vi "Should Stop.vi"(7 "Actor in":refnum<class "Actor.lvclass">, 8 "Error in":errorcluster, 10 "Msg Output":refnum<class "Msg Output.lvclass">) -> (0 "Error out":errorcluster, 2 "Stop":bool, 5 "Actor out":refnum<class "Actor.lvclass">)   [LabVIEW 2020, in "jettl.lvlib"]
uses:
  jettl.lvlib
  Actor/Actor.lvclass
  Msg Output/Msg Output.lvclass
  Msg/Msg.lvclass
  Teardown Location.ctl
  Stop jettl Msg/Stop/Call.vi
  Attributes/Attributes.lvclass
  Transport/Transport.lvclass
  Stop jettl Msg/Stop/Stop.lvlib
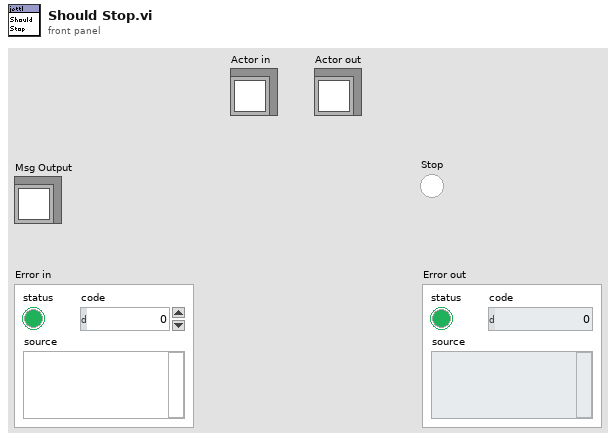
[diagram p1: front panel]
types:
  T1 = typedef "jettl.lvlib/Teardown Location.ctl" = enum16{"Starting", "Should Stop"}
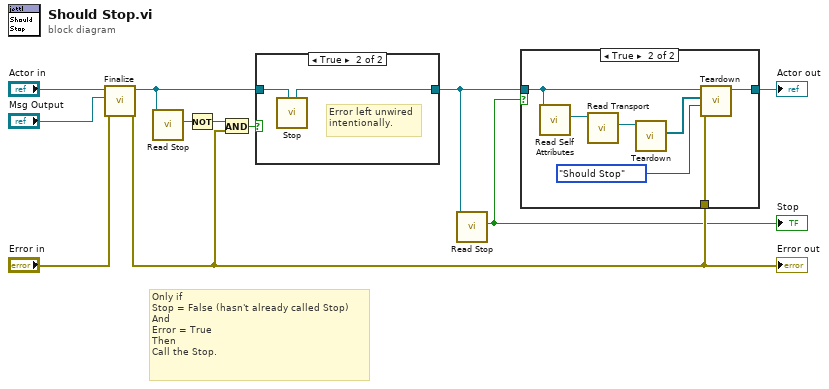
[diagram p0: block diagram]
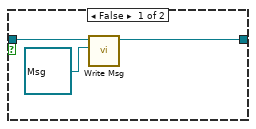
[diagram p3: hidden frame]
diagram:
  # "Only if\nStop = False (hasn't already called Stop)\nAnd\nError = True\nThen\nCall the Stop."
  n1 = call-dynamic "Finalize.vi"("Error in"="Error in", "Msg Output"="Msg Output", "Actor in"="Actor in") -> ("Error out"=w2:errorcluster, "Actor out"=w6:refnum<class "Actor.lvclass">)  [unwired: 7 in]
  "Error out" <- w2
  n2 = call-dynamic "Read Stop.vi"("Actor in"=w6) -> ("Stop"=w7:bool)  [unwired: 10 in]
  n3 = Not(x=w7) -> (.not. x?=w9:bool)
  n4 = And(x=w9, y=w2) -> (x .and. y?=w8:bool)
  n5 = case shown="True" w8 {
    tunnel: [w12 w13] -> w5
    tunnel: w6 -> [w12 w14]
    frame False {
    }
    frame True {
      # "Error left unwired intentionally."
      n6 = call-poly "Stop.vi"("Actor in"=w14) -> ("Actor out"=w13:refnum<class "Actor.lvclass">)  [unwired: 9 in, 1 out]
    }
  }
  n7 = call-dynamic "Read Stop.vi"("Actor in"=w5) -> ("Stop"=w1:bool)  [unwired: 10 in]
  "Stop" <- w1
  n8 = case shown="True" w1 {
    tunnel: w5 -> [w17 w20]
    tunnel: [w15 w19] -> w3
    tunnel: w2 -> [_ w18]
    frame False {
      n9 = call-dynamic "Write Msg.vi"("Msg"=refnum<class "Msg.lvclass"> refnum, "Actor in"=w17) -> ("Actor out"=w15:refnum<class "Actor.lvclass">)  [unwired: 9 in]
    }
    frame True {
      n10 = call-dynamic "Read Self Attributes.vi"("Actor in"=w20) -> ("Self Attributes"=w24:refnum<class "Attributes.lvclass">)  [unwired: 10 in]
      n11 = call-dynamic "Read Transport.vi"("Attributes in"=w24) -> ("Transport"=w23:refnum<class "Transport.lvclass">)  [unwired: 10 in]
      n12 = call-dynamic "Teardown.vi"("Transport in"=w23) -> ("Unheard Msgs"=w22:refnum<class "Msg.lvclass">[])  [unwired: 10 in]
      n13 = call-dynamic "Teardown.vi"("Error in"=w18, "Teardown Location"=Teardown_Location."Should Stop", "Unheard Msgs"=w22, "Actor in"=w20) -> ("Actor out"=w19:refnum<class "Actor.lvclass">)  [unwired: 7 in]
    }
  }
  "Actor out" <- w3
